vi "Host.vi"() -> ()   [LabVIEW 2018]
uses:
  <vilib>/userdefined/High Color/nirio_resource_hc.ctl
  <vilib>/vision/Image Controls.llb/IMAQ Image.ctl
  <instrlib>/niDCPower/nidcpower.llb/niDCPower Measurement Type.ctl
  <vilib>/FPGAPlugInAG/PXI-7953R/niLvFpga_Open_PXI-7953R.vi
  <vilib>/rvi/interface/common/dynamic/niFpgaDynamicAddResources.vi
  <vilib>/FPGAPlugInAG/Dynamic/niLvFpga_Reset_Dynamic.vi
  <vilib>/FPGAPlugInAG/Dynamic/niLvFpga_Run_Dynamic.vi
  <vilib>/Utility/error.llb/Error Cluster From Error Code.vi
  <vilib>/rvi/errors/niLvFpgaAdjustHostInterfaceError.vi
  <vilib>/FPGAPlugInAG/Dynamic/niLvFpga_Abort_Dynamic.vi
  <vilib>/rvi/interface/nirviOpenFPGA/nirviOpenFPGA.xnode
  FPGA Bitfiles/PelengCMV_FPGATarget_Target_uVRL8nzenuo.lvbitx
  <vilib>/rvi/interface/nirviMethod/nirviMethod.xnode
  <vilib>/rvi/interface/nirviReadWriteControl/nirviReadWriteControl.xnode
  NiFpgaLv.dll
  <vilib>/rvi/interface/Simulation/niFpgaSimulationCallBeginRW.vi
  <vilib>/FPGAPlugInAG/Dynamic/niLvFpga_ReadFifo_Dynamic.vi
  <vilib>/rvi/errors/niLvFpgaMergeErrorWithErrorCode.vi
panel:
  out "Waveform Chart 5":dbl(graph)=0.01180592873577935
  out "Waveform Chart 9":dbl(graph)=0.0007963780968987442
  out "Waveform Chart 7":dbl(graph)=0.08153866285805537
  out "Waveform Chart 6":dbl(graph)=-0.0005376097362887471
  out "Waveform Chart 4":dbl(graph)=0.015373157020534491
  out "Waveform Chart 3":dbl(graph)=-0.010436971741611662
  out "Waveform Chart 2":dbl(graph)=-0.0003554571679595278
  out "Тнак, мс":dbl
  in  "ПРОВЕРКА СБОЕВ?":bool=TRUE
  in  "ПРИМЕЧАНИЕ":string
  in  "Frames":path=path "C:/VPL/LabView_PRJ/ПЕЛЕНГ_CMV4000/FRAMES"
  in  "Светлый (T)\nТемный (F)":bool
  in  "SAVE":bool
  out "ПОСЛЕДНИЙ СБОЙ":string
  in  "МАСКИРУЕМ":i32[](array[numeric])=[0, 1, 2, 3, 4, 5, 6, 7, 8, 9, 10, 11, 12, 13, 14, 15, 16, 17, 18, 19, 20, 21, 22, 23, 24, 25, 26, 27, 28, 29, 30, 31, 32, 33, 34, 35, 36, 37, 38, 39, 40, 41, 42, 43, 44, 45, 46, 47, 48, 49, 50, 51, 52, 53, 54, 55, 56, 57, 58, 59, 60, 61, 62, 63, 64, 65, 66, 67, 68, 69, 70, 71, 72, 73, 74, 75, 76, 77, 78, 79, 80, 81, 82, 83, 84, 85, 86, 87, 88, 89, 90, 91, 92, 93, 94, 95, 96, 97, 98, 99, 100, 101, 102, 103, 104, 105, 106, 107, 108, 109, 110, 111, 112, 113, 114, 115, 116, 117, 118, 119, 120, 121, 122, 123, 124, 125, -1, -1, 0, 0, 0, 0, 0, 0, 0, 0, 0, 0, 0, 0, 0, 0, 0, 0, 0, 0, 0, 0, 0, 0, 0, 0, 0, 0, 0, 0, 0, 0, 0, 0, 0, 0, 0, 0, 0, 0, 0, 0, 0, 0, 0, 0, 0, 0, 0, 0, 0, 0, 0, 0, 0, 0, 0, 0, 0, 0, 0, 0, 0, 0, 0, 0, 0, 0, 0, 0, 0, 0, 0, 0, 0, 0, 0, 0, 0, 0, 0, 0, 0, 0, 0, 0, 0, 0, 0, 0, 0, 0, 0, 0, 0, 0, 0, 0, 0, 0, 0, 0, 0, 0, 0, 0, 0, 0, 0, 0, 0, 0, 0, 0, 0, 0, 0, 0, 0, 0, 0, 0, 0, 0, 0, 0, 0, 0, 0, 0]
  in  "НАДО":bool
  out "GC":u16
  in  "Непрерывно":bool
  out "Image":T1(plugin-control)
  in  "1":u8=1
  in  "2":u8=2
  in  "REQ_2":u8=7
  in  "REQ_1":u8=2
  in  "-1_прием":i8=-1
  out "Записали адресов":u32
  in  "9_прием":i8=9
  out "SPI_OUT":bool[](array[boolean])
  out "COUNT":u16
  out "D1":bool[](array[boolean])
  out "CONTROL":bool[](array[boolean])
  out "D9":bool[](array[boolean])
  out "T, C":dbl
  out "СБОЙ":string="ОК"
  in  "Запись всех регистров":u16[](array[numeric])=[0, 0, 8, 0, 0, 0, 0, 0, 0, 0, 0, 0, 0, 0, 0, 0, 0, 0, 0, 0, 0, 0, 0, 0, 0, 0, 0, 0, 0, 0, 0, 0, 0, 0, 0, 0, 0, 0, 0, 1, 0, 4, 0, 8, 0, 0, 0, 0, 1, 0, 0, 1, 0, 0, 1, 1, 0, 8, 0, 0, 0, 0, 1, 0, 0, 1, 0, 0, 1, 1, 1, 0, 3, 20, 8, 8, 8, 0, 85, 0, 255, 255, 3, 8, 4, 1, 14, 12, 64, 96, 96, 64, 96, 96, 101, 106, 96, 96, 96, 96, 0, 0, 3, 60, 8, 8, 8, 8, 0, 1, 0, 1, 0, 1, 3, 0, 9, 8, 1, 0, 0, 1, 0, 98, 0, 67]
  in  "SEU":path=path "C:/VPL/LabView_PRJ/ПЕЛЕНГ_CMV4000/LOGS/SEU"
  out "Сбои":i32
  in  "SEL_Time, мс":u32=100
  out "REG_WR":bool
  out "SEL":bool
  in  "For FIFO":i32=64
  in  "32768":u32=32768
  in  "Получить кадр":bool
  in  "VDD33_selcur":dbl=0.25 caption="current limit" format="%_6p"
  out "VDD33":i32
  out "VDD33":bool
  in  "SIM_SEL":bool
  in  "Облучаем?":bool
  in  "VDD20_selcur":dbl=0.2750000000000001 caption="current limit" format="%_6p"
  in  "VDDPIX_selcur":dbl=0.25000000000000006 caption="current limit" format="%_6p"
  in  "VRES_H_selcur":dbl=0.075 caption="current limit" format="%_6p"
  out "VDD20":i32
  out "VDD20":bool
  out "VDDPIX":i32=1
  out "VDDPIX":bool
  out "VRES_H":i32
  out "VRES_H":bool
  in  "REC(3,3V)":dbl=3.3 caption="voltage level" format="%_6p"
  in  "VDD20":dbl=5.0 caption="voltage level" format="%_6p"
  in  "VRES_H":dbl=5.0 caption="voltage level" format="%_6p"
  in  "REC_curlim":dbl=0.1 caption="current limit" format="%_6p"
  in  "FPGA+REP_curlim":dbl=0.5 caption="current limit" format="%_6p"
  in  "VDD20_curlim":dbl=0.30000000000000004 caption="current limit" format="%_6p"
  in  "VDD33_curlim":dbl=0.3 caption="current limit" format="%_6p"
  in  "VRES_H_curlim":dbl=0.1 caption="current limit" format="%_6p"
  out "REC_cur":dbl caption="measurement" format="%_6g"
  out "FPGA+REP_cur":dbl caption="measurement" format="%_6g"
  out "VDD20_cur":dbl caption="measurement" format="%_6g"
  out "VDD33_cur":dbl caption="measurement" format="%_6g"
  out "VRES_H_cur":dbl caption="measurement" format="%_6g"
  in  "FPGA+REP(6V)":dbl=5.0 caption="voltage level" format="%_6p"
  in  "VDD33":dbl=5.0 caption="voltage level" format="%_6p"
  in  "VDDPIX":dbl=5.0 caption="voltage level" format="%_6p"
  in  "VDDPIX_curlim":dbl=0.30000000000000004 caption="current limit" format="%_6p"
  out "VDDPIX_cur":dbl caption="measurement" format="%_6g"
  in  "TH_RES_curlim":dbl=0.2 caption="current limit" format="%_6p"
  out "TH_RES_cur":dbl caption="measurement" format="%_6g"
  in  "TH_RES":dbl=-20.0 caption="voltage level" format="%_6p"
  in  "Грелка":bool
  in  "Питание":bool
  in  "Стоп":bool
  in  "REC_FPGA_TH":refnum<k15>="PXI1Slot4" caption="instrument handle"
  in  "PIX_20":refnum<k15>="PXI1Slot2" caption="instrument handle"
  in  "33_RES":refnum<k15>="PXI1Slot3" caption="instrument handle"
  in  "resource name":T2="RIO0"
  in  "SEL":path=path "C:/VPL/LabView_PRJ/ПЕЛЕНГ_CMV4000/LOGS/SEL"
  out "Номер образца":string="1"
  out "Температура":string="25"
  out "Data":u32[][](array[numeric])
  out "Image Out":T1
  out "СБОЙ!":bool
  # "ЧТОБЫ ЗАМАСКИРОВАТЬ, ПОМЕНЯЙ НОМЕР РЕГИСТРА НА -1"
  # "КАЖДОЕ ВЫКЛЮЧЕНИЕ СОПРОВОЖДАЕТСЯ 300МС ЗАДЕРЖКОЙ"
  # "43 регистр\n8 = 53мс\n15 = 100мс\n30 = 200мс\n76 = 500мс\n152 = 1000мс\n227 = 1500мс"
  # "ЕСЛИ ХОЧЕШЬ СНЯТЬ ПРИ РАЗНЫХ ВРЕМЕНАХ НАКОПЛЕНИЯ, ТО ОТКЛЮЧИ ПРОВЕРКУ РЕГИСТРОВ И МЕНЯЙ ЗНАЧЕНИЕ В РЕГСИРЕ 43!"
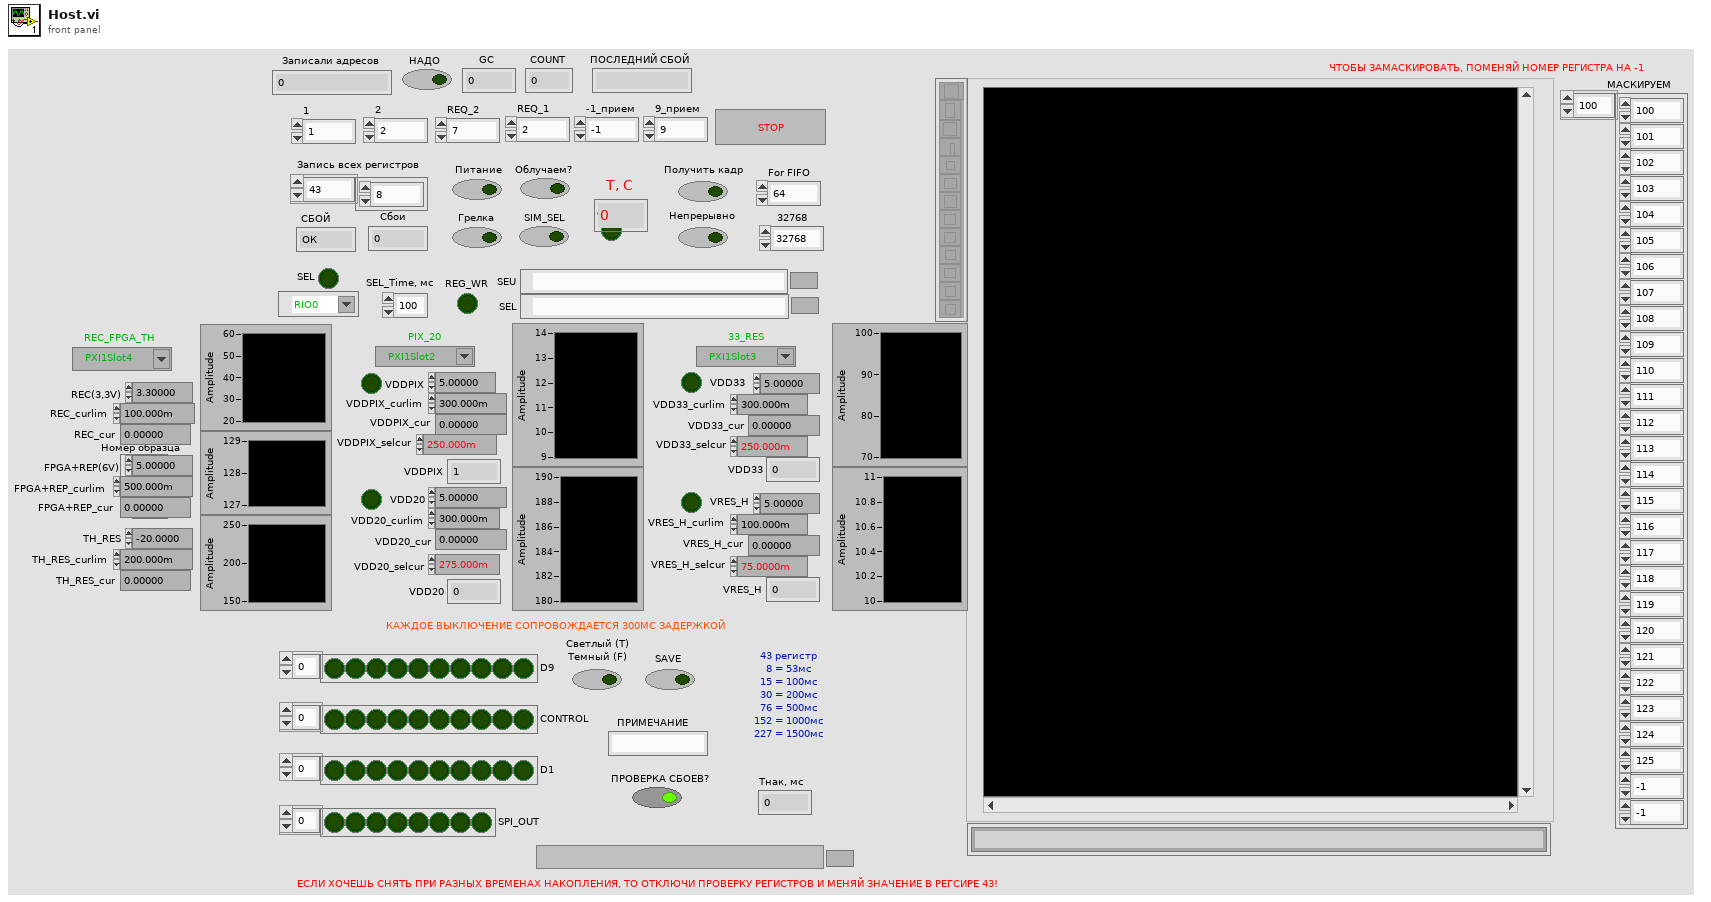
[diagram p1: front panel]
types:
  T1 = typedef "IMAQ Image.ctl" = refnum<image>
  T2 = typedef "nirio_resource_hc.ctl" = tag
  T3 = typedef "Image Type" = u32
  T4 = enum16{"open", "replace", "create", "open or create", "replace or create", "replace or create with confirmation"}
  T5 = typedef "niDCPower Measurement Type.ctl" = i32
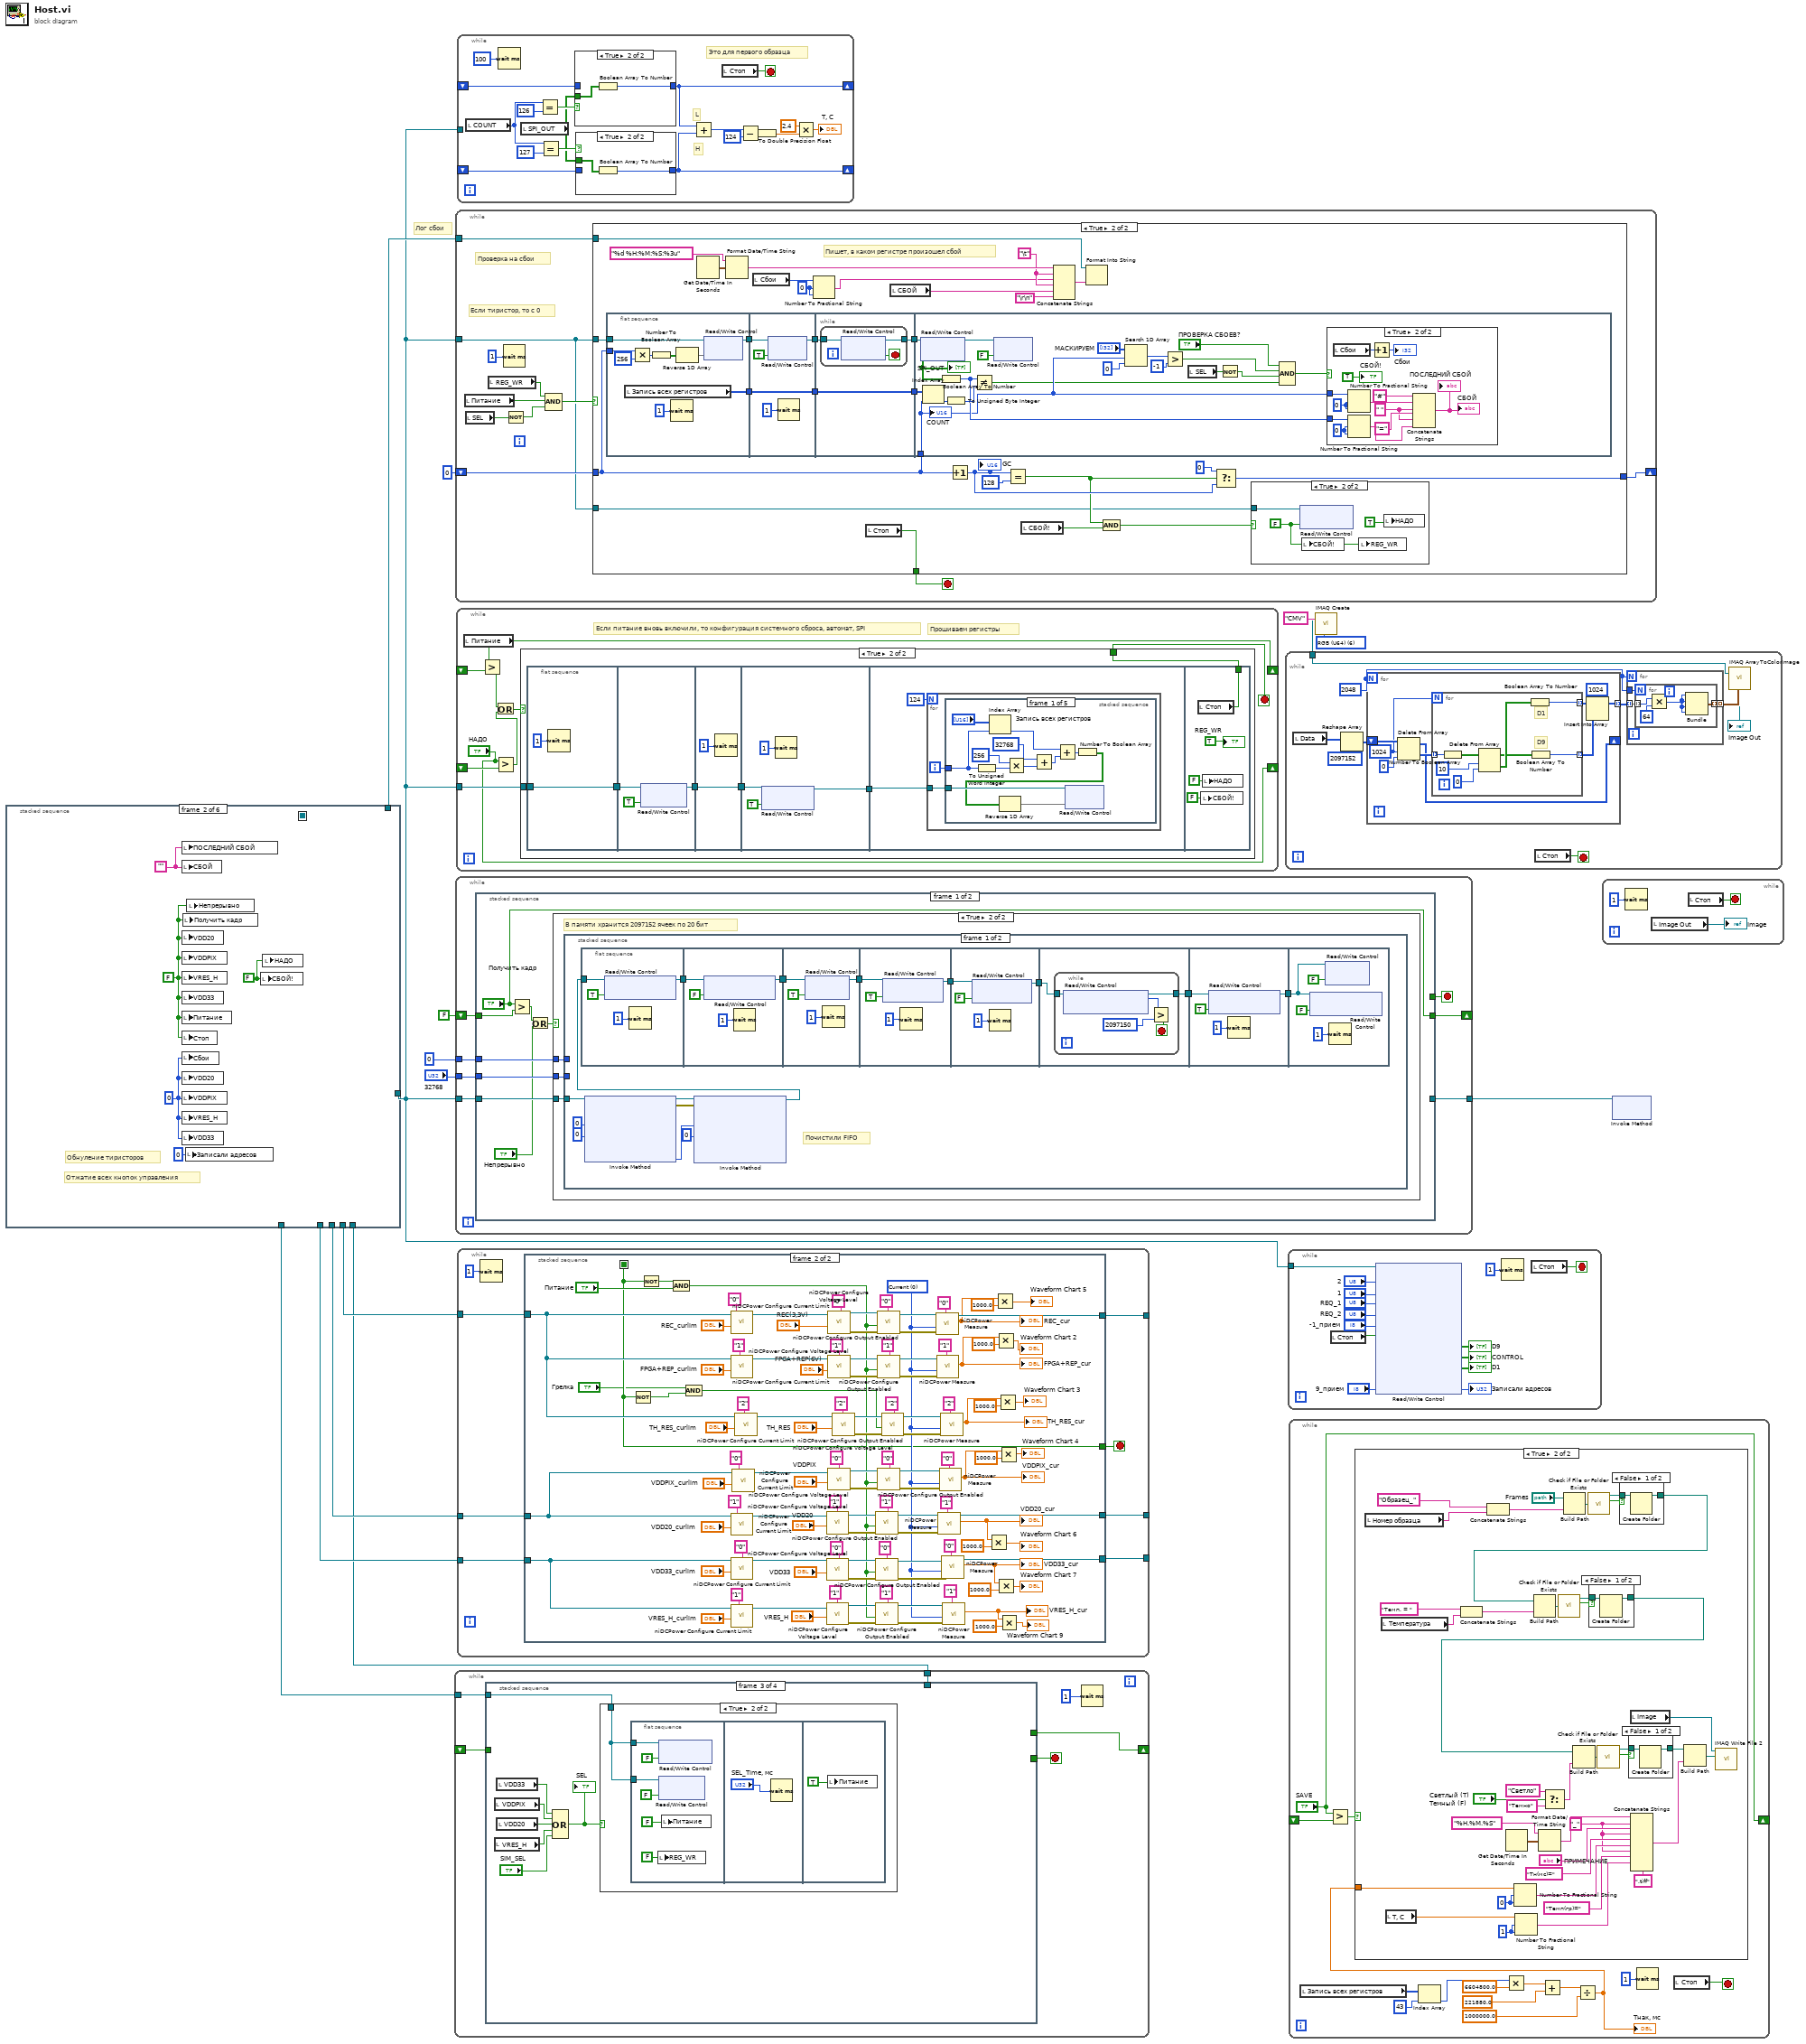
[diagram p0: block diagram]
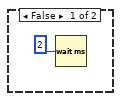
[diagram p8: hidden frame]
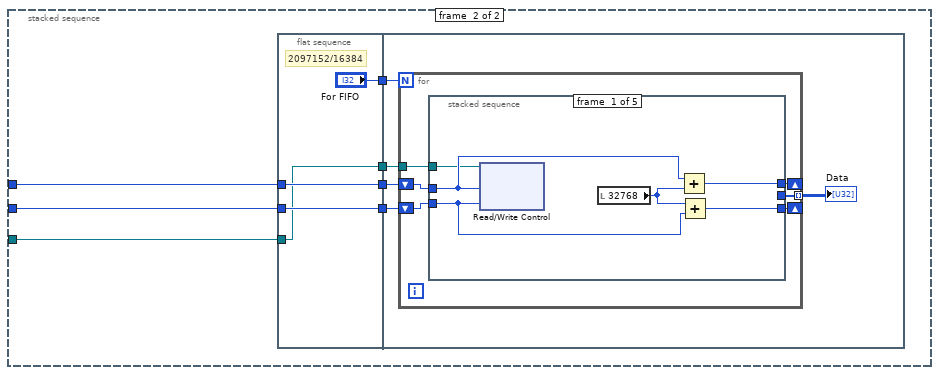
[diagram p9: hidden frame]
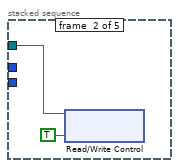
[diagram p10: hidden frame]
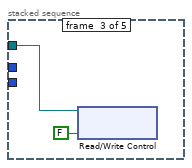
[diagram p11: hidden frame]
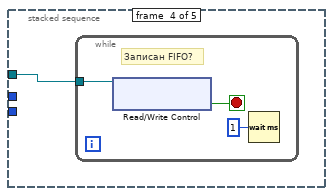
[diagram p12: hidden frame]
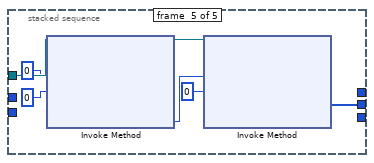
[diagram p13: hidden frame]
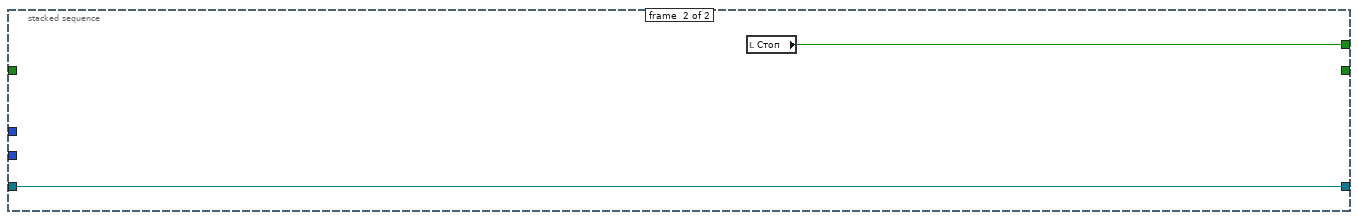
[diagram p14: hidden frame]
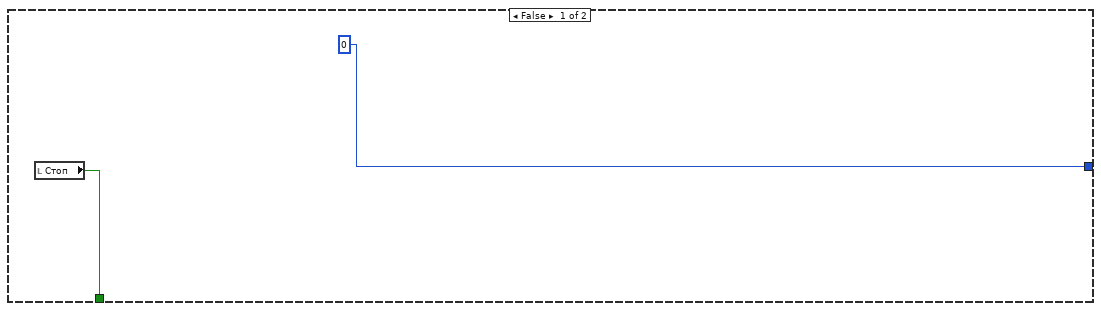
[diagram p15: hidden frame]
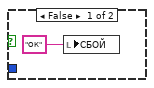
[diagram p17: hidden frame]
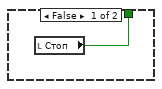
[diagram p18: hidden frame]
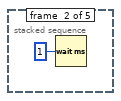
[diagram p19: hidden frame]
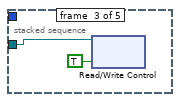
[diagram p20: hidden frame]
diagram:
  w3 = T3 6 items=["Grayscale (U8)", "Grayscale (I16)", "Grayscale (SGL)", "Complex (CSG)", "RGB (U32)", "HSL (U32)", "RGB (U64)"] ("Image Type")
  # "Лог сбои"
  n1 = stacked-sequence {
    seq-local: [_ _ _ _ w106 _] -> [_ _ _ _ _ w114]
    tunnel: [_ _ _ _ w106 _] -> w5
    tunnel: [_ _ _ _ _ w117] -> w13
    tunnel: [_ _ _ _ _ w116] -> w14
    tunnel: [_ _ _ _ _ w115] -> w15
    tunnel: [_ _ w29 _ _ _] -> w12
    tunnel: [_ _ _ _ w106 _] -> w10
    tunnel: [_ _ _ w68 _ _] -> w9
    frame #0 {
      n2 = call "Begin.vi"() -> ("Температура 2"=→"Температура":string, "Номер образца 2"=→"Номер образца":string)  [unwired: 10 in]
    }
    frame #1 {
      w22 = FALSE ("СБОЙ!")
      w19 = 0
      w20 = ""
      w21 = FALSE
      # "Обнуление тиристоров"
      # "Отжатие всех кнопок управления"
      n3 = local write "ПОСЛЕДНИЙ СБОЙ"(w20) -> ()
      n4 = local write "СБОЙ"(w20) -> ()
      n5 = local write "VDD20"(w21) -> ()
      n6 = local write "VDDPIX"(w21) -> ()
      n7 = local write "VRES_H"(w21) -> ()
      n8 = local write "VDD33"(w21) -> ()
      n9 = local write "Питание"(w21) -> ()
      n10 = local write "Стоп"(w21) -> ()
      n11 = local write "Сбои"(w19) -> ()
      n12 = local write "VDD20"(w19) -> ()
      n13 = local write "VDDPIX"(w19) -> ()
      n14 = local write "VRES_H"(w19) -> ()
      n15 = local write "VDD33"(w19) -> ()
      n16 = local write "Получить кадр"(w21) -> ()
      n17 = local write "Записали адресов"(u32 0 ("Записали адресов")) -> ()
      n18 = local write "Непрерывно"(w21) -> ()
      n19 = local write "СБОЙ!"(w22) -> ()
      n20 = local write "НАДО"(w22) -> ()
    }
    frame #2 {
      w32 = "\t"
      # "Инициализаци первой строки лога по токам"
      n21 = local read "Номер образца"() -> (w53:string)
      n22 = Build Path(base path="SEL", name or relative path=w53) -> (appended path=w55:path)
      n23 = Get Date/Time In Seconds() -> (seconds since 1Jan1904=w45:timestamp)
      n24 = call <vilib>:"Check if File or Folder Exists.vi"("path"=w55) -> ("file or folder exists?"=w56:bool, "dup path"=w57:path)  [unwired: 8 in, 1 out]
      n25 = Format Date/Time String(time format string (%c)="%d %H.%M.%S", seconds (now)=w45) -> (date/time string=w42:string)  [unwired: 1 in]
      n26 = case shown="False" w56 {
        tunnel: w57 -> [w66 w67]
        tunnel: [w65 w67] -> w51
        frame False {
          n27 = Create Folder(path (use dialog)=w66) -> (created path=w65:path)  [unwired: 2 in, 2 out]
        }
        frame True {
        }
      }
      n28 = local read "Температура"() -> (w50:string)
      n29 = Concatenate Strings(w42, ".xls" ("string")) -> (w40:string)
      n30 = Build Path(base path=w51, name or relative path=w50) -> (appended path=w31:path)
      n31 = call <vilib>:"Check if File or Folder Exists.vi"("path"=w31) -> ("file or folder exists?"=w30:bool, "dup path"=w52:path)  [unwired: 8 in, 1 out]
      n32 = case shown="False" w30 {
        tunnel: w52 -> [w63 w64]
        tunnel: [w62 w64] -> w39
        frame False {
          n33 = Create Folder(path (use dialog)=w63) -> (created path=w62:path)  [unwired: 2 in, 2 out]
        }
        frame True {
        }
      }
      n34 = Build Path(base path=w39, name or relative path=w40) -> (appended path=w43:path)
      n35 = Open/Create/Replace File(file path (use dialog)=w43, operation (0:open)=T4."open or create", access (0:read/write)=enum16{"read/write", "read-only", "write-only"}."read/write") -> (refnum out=w46:refnum<file>)  [unwired: 3 in, 2 out]
      n36 = case shown="True" TRUE {
        tunnel: w46 -> [w58 w61]
        tunnel: [w58 w59] -> w38
        frame False {
        }
        frame True {
          n37 = Set File Position(refnum=w61, from (0:start)=enum16{"start", "end", "current"}."end") -> (refnum out=w59:refnum<file>)  [unwired: 2 in, 1 out]
        }
      }
      n38 = Format Into String(initial string=w38, "Time" ("input 1"), w32, "VDD20_cur" ("input 1"), w32, "VDDPIX_cur" ("input 1"), w32, "VRES_H_cur" ("input 1"), w32, "VDD33_cur" ("input 1"), w32, "VDD20_sel" ("input 1"), w32, "VDDPIX_sel" ("input 1"), w32, "VRES_H_sel" ("input 1"), w32, "VDD33_sel" ("input 1"), w32, "Облучение" ("input 1"), "\r\n") -> (resulting string=w29:refnum<file>)  [unwired: 2 in, 1 out]
    }
    frame #3 {
      w77 = "\t"
      n39 = local read "Номер образца"() -> (w91:string)
      n40 = Build Path(base path="SEU", name or relative path=w91) -> (appended path=w93:path)
      n41 = Get Date/Time In Seconds() -> (seconds since 1Jan1904=w86:timestamp)
      n42 = call <vilib>:"Check if File or Folder Exists.vi"("path"=w93) -> ("file or folder exists?"=w94:bool, "dup path"=w95:path)  [unwired: 8 in, 1 out]
      n43 = Format Date/Time String(time format string (%c)="%d %H.%M.%S", seconds (now)=w86) -> (date/time string=w84:string)  [unwired: 1 in]
      n44 = case shown="False" w94 {
        tunnel: w95 -> [w104 w105]
        tunnel: [w103 w105] -> w89
        frame False {
          n45 = Create Folder(path (use dialog)=w104) -> (created path=w103:path)  [unwired: 2 in, 2 out]
        }
        frame True {
        }
      }
      n46 = local read "Температура"() -> (w88:string)
      n47 = Concatenate Strings(w84, ".xls" ("string")) -> (w83:string)
      n48 = Build Path(base path=w89, name or relative path=w88) -> (appended path=w80:path)
      n49 = call <vilib>:"Check if File or Folder Exists.vi"("path"=w80) -> ("file or folder exists?"=w79:bool, "dup path"=w90:path)  [unwired: 8 in, 1 out]
      n50 = case shown="False" w79 {
        tunnel: w90 -> [w101 w102]
        tunnel: [w100 w102] -> w82
        frame False {
          n51 = Create Folder(path (use dialog)=w101) -> (created path=w100:path)  [unwired: 2 in, 2 out]
        }
        frame True {
        }
      }
      n52 = Build Path(base path=w82, name or relative path=w83) -> (appended path=w85:path)
      n53 = Open/Create/Replace File(file path (use dialog)=w85, operation (0:open)=T4."open or create", access (0:read/write)=enum16{"read/write", "read-only", "write-only"}."read/write") -> (refnum out=w87:refnum<file>)  [unwired: 3 in, 2 out]
      n54 = case shown="True" TRUE {
        tunnel: w87 -> [w96 w99]
        tunnel: [w96 w97] -> w81
        frame False {
        }
        frame True {
          n55 = Set File Position(refnum=w99, from (0:start)=enum16{"start", "end", "current"}."end") -> (refnum out=w97:refnum<file>)  [unwired: 2 in, 1 out]
        }
      }
      n56 = Format Into String(initial string=w81, "Time" ("input 1"), w77, "Count" ("input 3"), w77, "#reg" ("input 5"), "\r\n") -> (resulting string=w68:refnum<file>)  [unwired: 2 in, 1 out]
    }
    frame #4 {
      n57 = xnode "Open FPGA VI Reference"("resource name"="resource name") -> ("FPGA VI Reference Out"=w111:refnum<k20>, "error out"=w109:errorcluster)  [unwired: 1 in]
      n58 = xnode "Invoke Method"("FPGA VI Reference In"=w111, "error in"=w109) -> ("FPGA VI Reference Out"=w108:refnum<k20>, "error out"=w110:errorcluster)
      n59 = xnode "Invoke Method"("FPGA VI Reference In"=w108, "error in"=w110) -> ("FPGA VI Reference Out"=w106:refnum<k20>)  [unwired: 1 in, 1 out]
    }
    frame #5 {
      w112 = FALSE ("SYS_RESET")
      n60 = xnode "Read/Write Control"("FPGA VI Reference In"=w114, "SYS_RESET"=w112, "Стоп"=w112, "Данные"=w112, "FRAME_REQ"=w112, "Конец анализа"=w112) -> ()  [unwired: 1 in, 2 out]
      n61 = local write "REG_WR"(FALSE ("Прошили регистры")) -> ()
      n62 = call <instrlib>:"niDCPower Initialize.vi"("resource name"="REC_FPGA_TH") -> ("error out"=w127:errorcluster, "instrument handle out"=w130:refnum<k15>)  [unwired: 3 in, 6 out]
      n63 = call <instrlib>:"niDCPower Initialize.vi"("resource name"="PIX_20") -> ("error out"=w128:errorcluster, "instrument handle out"=w131:refnum<k15>)  [unwired: 3 in, 6 out]
      n64 = call <instrlib>:"niDCPower Initialize.vi"("resource name"="33_RES") -> ("error out"=w129:errorcluster, "instrument handle out"=w132:refnum<k15>)  [unwired: 3 in, 6 out]
      n65 = call <instrlib>:"niDCPower Configure Voltage Level.vi"("error in (no error)"=w127, "voltage level"=0.0, "channel name"="0,1,2", "instrument handle"=w130) -> ("instrument handle out"=w115:refnum<k15>)  [unwired: 6 in, 1 out]
      n66 = call <instrlib>:"niDCPower Configure Voltage Level.vi"("error in (no error)"=w128, "voltage level"=0.0, "channel name"="0,1", "instrument handle"=w131) -> ("instrument handle out"=w116:refnum<k15>)  [unwired: 6 in, 1 out]
      n67 = call <instrlib>:"niDCPower Configure Voltage Level.vi"("error in (no error)"=w129, "voltage level"=0.0, "channel name"="0,1", "instrument handle"=w132) -> ("instrument handle out"=w117:refnum<k15>)  [unwired: 6 in, 1 out]
    }
  }
  n68 = while {
    tunnel: w12 -> [w137]
    shift-right: [w136] -> _
    shift-left: _ -> [w135]
    tunnel: w10 -> [w133]
    stop <- w134 stop-if-true
    n69 = stacked-sequence {
      tunnel: w137 -> [_ w200 _ _]
      tunnel: [w141 _ _ _] -> w136
      tunnel: w135 -> [w139 _ _ _]
      tunnel: [_ _ _ w224] -> w134
      tunnel: w133 -> [_ _ w207 w222]
      frame #0 {
        # "Проверка токов на тиристоры"
        n70 = local read "Питание"() -> (w141:bool)
        n71 = flat-sequence {
          tunnel: w140 -> [w142]
          frame #0 {
            n72 = case shown="True" w142 {
              frame False {
              }
              frame True {
                n73 = Wait (ms)(milliseconds to wait=u32 300) -> ()  [unwired: 1 out]
              }
            }
          }
          frame #1 {
            n74 = local read "VDD33_cur"() -> (w144:dbl)
            n75 = local read "VRES_H_cur"() -> (w149:dbl)
            n76 = local read "VDDPIX_cur"() -> (w152:dbl)
            n77 = local read "VDD20_cur"() -> (w155:dbl)
            n78 = Greater?(x=w144, y="VDD33_selcur") -> (0:w146:bool)
            "VDD33" <- w146
            n79 = Greater?(x=w149, y="VRES_H_selcur") -> (0:w147:bool)
            "VRES_H" <- w147
            n80 = Greater?(x=w155, y="VDD20_selcur") -> (0:w153:bool)
            "VDD20" <- w153
            n81 = Greater?(x=w152, y="VDDPIX_selcur") -> (0:w150:bool)
            "VDDPIX" <- w150
            n82 = case shown="True" w146 {
              frame False {
              }
              frame True {
                n83 = local read "VDD33"() -> (w157:i32)
                n84 = Increment(x=w157) -> (x+1=→"VDD33":i32)
              }
            }
            n85 = case shown="True" w153 {
              frame False {
              }
              frame True {
                n86 = local read "VDD20"() -> (w163:i32)
                n87 = Increment(x=w163) -> (x+1=→"VDD20":i32)
              }
            }
            n88 = case shown="True" w150 {
              frame False {
              }
              frame True {
                n89 = local read "VDDPIX"() -> (w160:i32)
                n90 = Increment(x=w160) -> (x+1=→"VDDPIX":i32)
              }
            }
            n91 = case shown="True" w147 {
              frame False {
              }
              frame True {
                n92 = local read "VRES_H"() -> (w159:i32)
                n93 = Increment(x=w159) -> (x+1=→"VRES_H":i32)
              }
            }
          }
        }
        n94 = Greater?(x=w141, y=w139) -> (0:w140:bool)
      }
      frame #1 {
        w166 = i16 2 ("precision (6)")
        w185 = i16 0 ("width (-)")
        w190 = i16 3 ("width (-)")
        w169 = "\t"
        n95 = local read "VDDPIX_cur"() -> (w188:dbl)
        n96 = local read "VRES_H_cur"() -> (w187:dbl)
        n97 = local read "VDD20_cur"() -> (w189:dbl)
        n98 = local read "VDD33_cur"() -> (w186:dbl)
        n99 = local read "VDDPIX"() -> (w183:i32)
        n100 = local read "VRES_H"() -> (w182:i32)
        n101 = local read "VDD20"() -> (w184:i32)
        n102 = local read "VDD33"() -> (w181:i32)
        n103 = Number To Fractional String(number=w189, width (-)=w190, precision (6)=w190) -> (F-format string=w180:string)  [unwired: 1 in]
        n104 = Number To Fractional String(number=w188, width (-)=w190, precision (6)=w190) -> (F-format string=w179:string)  [unwired: 1 in]
        n105 = Number To Fractional String(number=w187, width (-)=w190, precision (6)=w190) -> (F-format string=w178:string)  [unwired: 1 in]
        n106 = Number To Fractional String(number=w186, width (-)=w190, precision (6)=w190) -> (F-format string=w177:string)  [unwired: 1 in]
        n107 = Number To Fractional String(number=w184, width (-)=w185, precision (6)=w185) -> (F-format string=w176:string)  [unwired: 1 in]
        n108 = Number To Fractional String(number=w183, width (-)=w185, precision (6)=w185) -> (F-format string=w175:string)  [unwired: 1 in]
        n109 = Number To Fractional String(number=w182, width (-)=w185, precision (6)=w185) -> (F-format string=w174:string)  [unwired: 1 in]
        n110 = Number To Fractional String(number=w181, width (-)=w185, precision (6)=w185) -> (F-format string=w173:string)  [unwired: 1 in]
        n111 = Get Date/Time In Seconds() -> (seconds since 1Jan1904=w205:timestamp)
        n112 = Format Date/Time String(time format string (%c)="%d %H:%M:%S:%3u", seconds (now)=w205) -> (date/time string=w191:string)  [unwired: 1 in]
        n113 = local read "VDD33"() -> (w196:bool)
        n114 = local read "VDDPIX"() -> (w195:bool)
        n115 = local read "VDD20"() -> (w194:bool)
        n116 = local read "VRES_H"() -> (w193:bool)
        n117 = local read "SIM_SEL"() -> (w192:bool)
        n118 = Compound Arithmetic op=OR(w196, w195, w194, w193, w192) -> (w172:bool)
        n119 = Select(t="О", s="Облучаем?", f="") -> (s? t:f=w171:string)
        n120 = Select(t="!!!", s=w172, f="") -> (s? t:f=w170:string)
        n121 = local read "T, C"() -> (w167:dbl)
        n122 = Number To Fractional String(number=w167, width (-)=w166, precision (6)=w166) -> (F-format string=w165:string)  [unwired: 1 in]
        n123 = Concatenate Strings(w191, w169, w180, w169, w179, w169, w178, w169, w177, w169, w176, w169, w175, w169, w174, w169, w173, w169, w171, w169, w170, w169, "Т = ", w165, "\r\n") -> (w204:string)
        n124 = Format Into String(initial string=w200, w204) -> ()  [unwired: 2 in, 2 out]
      }
      frame #2 {
        n125 = local read "VDDPIX"() -> (w211:bool)
        n126 = local read "VRES_H"() -> (w209:bool)
        n127 = local read "VDD33"() -> (w212:bool)
        n128 = local read "VDD20"() -> (w210:bool)
        n129 = Compound Arithmetic op=OR(w212, w211, w210, w209, "SIM_SEL") -> (w206:bool)
        "SEL" <- w206
        n130 = case shown="True" w206 {
          tunnel: w207 -> [_ w213]
          frame False {
          }
          frame True {
            n131 = flat-sequence {
              tunnel: w213 -> [w218]
              tunnel: w213 -> [w217]
              frame #0 {
                n132 = local write "REG_WR"(FALSE ("SYS_RESET")) -> ()
                n133 = xnode "Read/Write Control"("FPGA VI Reference In"=w217, "Автомат"=FALSE ("SYS_RESET")) -> ()  [unwired: 1 in, 2 out]
                n134 = xnode "Read/Write Control"("FPGA VI Reference In"=w218, "SYS_RESET"=FALSE) -> ()  [unwired: 1 in, 2 out]
                n135 = local write "Питание"(FALSE ("SYS_RESET")) -> ()
              }
              frame #1 {
                n136 = Wait (ms)(milliseconds to wait="SEL_Time, мс") -> ()  [unwired: 1 out]
              }
              frame #2 {
                n137 = local write "Питание"(TRUE ("SYS_RESET")) -> ()
              }
            }
          }
        }
      }
      frame #3 {
        n138 = local read "Питание"() -> (w223:bool)
        n139 = case shown="False" w223 {
          tunnel: w222 -> [w226 _]
          frame False {
            w225 = FALSE
            n140 = xnode "Read/Write Control"("FPGA VI Reference In"=w226, "SYS_RESET"=w225) -> ()  [unwired: 1 in, 2 out]
            n141 = xnode "Read/Write Control"("FPGA VI Reference In"=w226, "Автомат"=w225) -> ()  [unwired: 1 in, 2 out]
            n142 = local write "REG_WR"(w225) -> ()
          }
          frame True {
          }
        }
        n143 = local read "Стоп"() -> (w224:bool)
      }
    }
    n144 = Wait (ms)(milliseconds to wait=u32 1) -> ()  [unwired: 1 out]
  }
  n145 = while {
    tunnel: w5 -> [w227]
    tunnel: w9 -> [w229]
    shift-right: [w230] -> _
    shift-left: u16 0 -> [w231]
    stop <- w228 stop-if-true
    # "Проверка на сбои"
    # "Если тиристор, то с 0"
    n146 = local read "Питание"() -> (w236:bool)
    n147 = local read "SEL"() -> (w234:bool)
    n148 = local read "REG_WR"() -> (w237:bool)
    n149 = Wait (ms)(milliseconds to wait=u32 1) -> ()  [unwired: 1 out]
    n150 = Not(x=w234) -> (.not. x?=w233:bool)
    n151 = Compound Arithmetic op=AND(w237, w236, w233) -> (w235:bool)
    n152 = case shown="True" w235 {
      tunnel: w231 -> [_ w261]
      tunnel: [u8 0 w266] -> w230
      tunnel: w227 -> [_ w265]
      tunnel: w229 -> [_ w254]
      tunnel: [w238 w245] -> w228
      tunnel: w227 -> [_ w240]
      frame False {
        n153 = local read "Стоп"() -> (w238:bool)
      }
      frame True {
        w250 = i16 0 ("width (-)")
        w252 = "\t"
        # "Пишет, в каком регистре произошел сбой"
        n154 = flat-sequence {
          tunnel: w261 -> [w279]
          tunnel: w265 -> [w274]
          tunnel: [w273] -> w264
          tunnel: [w272] -> w258
          tunnel: w264 -> [w284]
          tunnel: [w281] -> w263
          tunnel: [w280] -> w259
          tunnel: w258 -> [w280]
          tunnel: w263 -> [w287]
          tunnel: [w286] -> w262
          tunnel: [w285] -> w260
          tunnel: w259 -> [w285]
          tunnel: w262 -> [w309]
          tunnel: w261 -> [w297]
          tunnel: w260 -> [w308]
          frame #0 {
            n155 = local read "Запись всех регистров"() -> (w272:u16[])
            n156 = Multiply(x=w279, y=u16 256) -> (x*y=w276:u16)
            n157 = Number To Boolean Array(number=w276) -> (Boolean array=w277:bool[])
            n158 = Wait (ms)(milliseconds to wait=u32 1) -> ()  [unwired: 1 out]
            n159 = Reverse 1D Array(array=w277) -> (reversed array=w275:bool[])
            n160 = xnode "Read/Write Control"("FPGA VI Reference In"=w274, "SPI_IN"=w275) -> ("FPGA VI Reference Out"=w273:refnum<k20>)  [unwired: 1 in, 1 out]
          }
          frame #1 {
            n161 = xnode "Read/Write Control"("FPGA VI Reference In"=w284, "SPI"=TRUE) -> ("FPGA VI Reference Out"=w281:refnum<k20>)  [unwired: 1 in, 1 out]
            n162 = Wait (ms)(milliseconds to wait=u32 1) -> ()  [unwired: 1 out]
          }
          frame #2 {
            n163 = while {
              tunnel: w287 -> [w290]
              tunnel: [w288] -> w286
              stop <- w289 stop-if-true
              n164 = xnode "Read/Write Control"("FPGA VI Reference In"=w290) -> ("FPGA VI Reference Out"=w288:refnum<k20>, "SPI_OFF"=w289:bool)  [unwired: 1 in, 1 out]
            }
          }
          frame #3 {
            n165 = xnode "Read/Write Control"("FPGA VI Reference In"=w309) -> ("FPGA VI Reference Out"=w304:refnum<k20>, "SPI_OUT"=w307:bool[])  [unwired: 1 in, 1 out]
            "SPI_OUT" <- w307
            n166 = Index Array(array=w308, index=w297) -> (element=w306:u16)
            n167 = Boolean Array To Number(Boolean array=w307) -> (number=w302:u8)
            n168 = To Unsigned Byte Integer(number=w306) -> (unsigned 8bit integer=w305:u8)
            n169 = Not Equal?(x=w302, y=w305) -> (x != y?=w292:bool)
            n170 = xnode "Read/Write Control"("FPGA VI Reference In"=w304, "SPI"=FALSE) -> ()  [unwired: 1 in, 2 out]
            n171 = Search 1D Array(1D array="МАСКИРУЕМ", element=w297, start index (0)=0) -> (index of element=w298:i32)
            n172 = Greater?(x=w298, y=-1) -> (0:w294:bool)
            n173 = local read "SEL"() -> (w296:bool)
            n174 = Not(x=w296) -> (.not. x?=w293:bool)
            n175 = Compound Arithmetic op=AND("ПРОВЕРКА СБОЕВ?", w294, w293, w292) -> (w291:bool)
            n176 = case shown="True" w291 {
              tunnel: w297 -> [_ w315]
              tunnel: w302 -> [_ w314]
              frame False {
                n177 = local write "СБОЙ"("ОК" ("Где сбой")) -> ()
              }
              frame True {
                w311 = " " ("string")
                w320 = i16 0 ("width (-)")
                w321 = i16 0 ("width (-)")
                n178 = local read "Сбои"() -> (w323:i32)
                n179 = Number To Fractional String(number=w315, width (-)=w321, precision (6)=w321) -> (F-format string=w318:string)  [unwired: 1 in]
                n180 = Number To Fractional String(number=w314, width (-)=w320, precision (6)=w320) -> (F-format string=w312:string)  [unwired: 1 in]
                n181 = Increment(x=w323) -> (x+1=→"Сбои":i32)
                n182 = Concatenate Strings("#" ("string"), w318, w311, "=" ("string"), w311, w312) -> (→"СБОЙ" →"ПОСЛЕДНИЙ СБОЙ":string)
                "СБОЙ!" <- TRUE ("СБОЙ!")
              }
            }
            "COUNT" <- w297
          }
        }
        n183 = Get Date/Time In Seconds() -> (seconds since 1Jan1904=w257:timestamp)
        n184 = Format Date/Time String(time format string (%c)="%d %H:%M:%S:%3u", seconds (now)=w257) -> (date/time string=w255:string)  [unwired: 1 in]
        n185 = local read "Сбои"() -> (w249:i32)
        n186 = Number To Fractional String(number=w249, width (-)=w250, precision (6)=w250) -> (F-format string=w248:string)  [unwired: 1 in]
        n187 = local read "Стоп"() -> (w245:bool)
        n188 = local read "СБОЙ"() -> (w247:string)
        n189 = Increment(x=w261) -> (x+1=w246:u16)
        "GC" <- w246
        n190 = Equal?(x=w246, y=u16 128) -> (x = y?=w243:bool)
        n191 = local read "СБОЙ!"() -> (w242:bool)
        n192 = Concatenate Strings(w255, w252, w248, w252, w247, "\r\n") -> (w253:string)
        n193 = Format Into String(initial string=w254, w253) -> ()  [unwired: 2 in, 2 out]
        n194 = And(x=w243, y=w242) -> (x .and. y?=w241:bool)
        n195 = Select(t=u16 0, s=w243, f=w246) -> (s? t:f=w266:u16)
        n196 = case shown="True" w241 {
          tunnel: w240 -> [_ w270]
          frame False {
          }
          frame True {
            w269 = FALSE ("SYS_RESET")
            n197 = xnode "Read/Write Control"("FPGA VI Reference In"=w270, "SYS_RESET"=w269) -> ()  [unwired: 1 in, 2 out]
            n198 = local write "СБОЙ!"(w269) -> ()
            n199 = local write "REG_WR"(w269) -> ()
            n200 = local write "НАДО"(TRUE ("НАДО")) -> ()
          }
        }
      }
    }
  }
  n201 = while {
    tunnel: w5 -> [w330]
    tunnel: [w329] -> w11
    tunnel: "32768" -> [w328]
    tunnel: u32 0 -> [w326]
    shift-right: [w324] -> _
    shift-left: FALSE ("Получить кадр") -> [w325]
    stop <- w327 stop-if-true
    n202 = stacked-sequence {
      tunnel: w330 -> [w337 w437]
      tunnel: [_ w437] -> w329
      tunnel: w328 -> [w338 _]
      tunnel: [_ w436] -> w327
      tunnel: w326 -> [w336 _]
      tunnel: w325 -> [w335 _]
      tunnel: ["Получить кадр" _] -> w324
      frame #0 {
        n203 = Greater?(x="Получить кадр", y=w335) -> (0:w334:bool)
        n204 = Or(x=w334, y="Непрерывно") -> (x .or. y?=w332:bool)
        n205 = case shown="True" w332 {
          tunnel: w337 -> [_ w342]
          tunnel: w338 -> [_ w341]
          tunnel: w336 -> [_ w340]
          frame False {
            n206 = Wait (ms)(milliseconds to wait=u32 2) -> ()  [unwired: 1 out]
          }
          frame True {
            # "В памяти хранится 2097152 ячеек по 20 бит"
            n207 = stacked-sequence {
              tunnel: w342 -> [w346 w399]
              tunnel: w341 -> [_ w395]
              tunnel: w340 -> [_ w397]
              frame #0 {
                # "Почистили FIFO"
                n208 = flat-sequence {
                  tunnel: w345 -> [w361]
                  tunnel: [w360] -> w349
                  tunnel: [w365] -> w350
                  tunnel: w349 -> [w364]
                  tunnel: w350 -> [w367]
                  tunnel: [w366] -> w348
                  tunnel: [w371] -> w351
                  tunnel: w348 -> [w370]
                  tunnel: w351 -> [w375]
                  tunnel: [w374] -> w347
                  tunnel: w347 -> [w379]
                  tunnel: [w378] -> w344
                  tunnel: w344 -> [w386]
                  tunnel: [w385] -> w343
                  tunnel: w343 -> [w389]
                  frame #0 {
                    n209 = xnode "Read/Write Control"("FPGA VI Reference In"=w361, "Конец анализа"=TRUE) -> ("FPGA VI Reference Out"=w360:refnum<k20>)  [unwired: 1 in, 1 out]
                    n210 = Wait (ms)(milliseconds to wait=u32 1) -> ()  [unwired: 1 out]
                  }
                  frame #1 {
                    n211 = xnode "Read/Write Control"("FPGA VI Reference In"=w364, "Конец анализа"=FALSE) -> ("FPGA VI Reference Out"=w365:refnum<k20>)  [unwired: 1 in, 1 out]
                    n212 = Wait (ms)(milliseconds to wait=u32 1) -> ()  [unwired: 1 out]
                  }
                  frame #2 {
                    n213 = xnode "Read/Write Control"("FPGA VI Reference In"=w367, "Данные"=TRUE) -> ("FPGA VI Reference Out"=w366:refnum<k20>)  [unwired: 1 in, 1 out]
                    n214 = Wait (ms)(milliseconds to wait=u32 1) -> ()  [unwired: 1 out]
                  }
                  frame #3 {
                    n215 = xnode "Read/Write Control"("FPGA VI Reference In"=w370, "FRAME_REQ"=TRUE ("Данные")) -> ("FPGA VI Reference Out"=w371:refnum<k20>)  [unwired: 1 in, 1 out]
                    n216 = Wait (ms)(milliseconds to wait=u32 1) -> ()  [unwired: 1 out]
                  }
                  frame #4 {
                    n217 = xnode "Read/Write Control"("FPGA VI Reference In"=w375, "FRAME_REQ"=FALSE ("Данные")) -> ("FPGA VI Reference Out"=w374:refnum<k20>)  [unwired: 1 in, 1 out]
                    n218 = Wait (ms)(milliseconds to wait=u32 1) -> ()  [unwired: 1 out]
                  }
                  frame #5 {
                    n219 = while {
                      tunnel: w379 -> [w381]
                      tunnel: [w380] -> w378
                      stop <- w384 stop-if-true
                      n220 = xnode "Read/Write Control"("FPGA VI Reference In"=w381) -> ("FPGA VI Reference Out"=w380:refnum<k20>, "Записали адресов"=w383:u32)  [unwired: 1 in, 1 out]
                      n221 = Greater?(x=w383, y=u32 2097150) -> (0:w384:bool)
                    }
                  }
                  frame #6 {
                    n222 = xnode "Read/Write Control"("FPGA VI Reference In"=w386, "Конец анализа"=TRUE ("Данные")) -> ("FPGA VI Reference Out"=w385:refnum<k20>)  [unwired: 1 in, 1 out]
                    n223 = Wait (ms)(milliseconds to wait=u32 1) -> ()  [unwired: 1 out]
                  }
                  frame #7 {
                    n224 = xnode "Read/Write Control"("FPGA VI Reference In"=w389, "Конец анализа"=FALSE ("Данные")) -> ()  [unwired: 1 in, 2 out]
                    n225 = xnode "Read/Write Control"("FPGA VI Reference In"=w389, "Данные"=FALSE) -> ()  [unwired: 1 in, 2 out]
                    n226 = Wait (ms)(milliseconds to wait=u32 1) -> ()  [unwired: 1 out]
                  }
                }
                n227 = xnode "Invoke Method"("FPGA VI Reference In"=w346, "Number of Elements"=u32 0, "Timeout (ms)"=0) -> ("FPGA VI Reference Out"=w357:refnum<k20>, "error out"=w356:errorcluster, "Elements Remaining"=w355:u32)  [unwired: 1 in, 1 out]
                n228 = xnode "Invoke Method"("FPGA VI Reference In"=w357, "error in"=w356, "Number of Elements"=w355, "Timeout (ms)"=0) -> ("FPGA VI Reference Out"=w345:refnum<k20>)  [unwired: 3 out]
              }
              frame #1 {
                n229 = flat-sequence {
                  tunnel: w399 -> [w400]
                  tunnel: [w403] -> w398
                  tunnel: w397 -> [w403]
                  tunnel: [w402] -> w396
                  tunnel: w395 -> [w402]
                  tunnel: ["For FIFO"] -> w394
                  tunnel: [w400] -> w393
                  tunnel: w398 -> [w408]
                  tunnel: w396 -> [w407]
                  tunnel: w394 -> [w406]
                  tunnel: w393 -> [w405]
                  frame #0 {
                    # "2097152/16384"
                  }
                  frame #1 {
                    n230 = for {
                      N: w406 -> [_]
                      shift-right: [w412] -> _
                      shift-left: w408 -> [w414]
                      shift-right: [w411] -> _
                      shift-left: w407 -> [w413]
                      tunnel: w405 -> [w410]
                      tunnel: [w409] -> w404 mode=indexing
                      n231 = stacked-sequence {
                        tunnel: [_ _ _ _ w433] -> w409
                        tunnel: [w420 _ _ _ _] -> w412
                        tunnel: [w419 _ _ _ _] -> w411
                        tunnel: w414 -> [w416 _ _ _ _]
                        tunnel: w413 -> [w417 _ _ _ _]
                        tunnel: w410 -> [w415 w421 w423 w425 w432]
                        frame #0 {
                          n232 = xnode "Read/Write Control"("FPGA VI Reference In"=w415, "Нач_адр"=w416, "Кон_адр"=w417) -> ()  [unwired: 1 in, 2 out]
                          n233 = local read "32768"() -> (w418:u32)
                          n234 = Add(x=w416, y=w418) -> (x+y=w420:u32)
                          n235 = Add(x=w418, y=w417) -> (x+y=w419:u32)
                        }
                        frame #1 {
                          n236 = xnode "Read/Write Control"("FPGA VI Reference In"=w421, "Кадр на ПК"=TRUE ("HOST")) -> ()  [unwired: 1 in, 2 out]
                        }
                        frame #2 {
                          n237 = xnode "Read/Write Control"("FPGA VI Reference In"=w423, "Кадр на ПК"=FALSE ("HOST")) -> ()  [unwired: 1 in, 2 out]
                        }
                        frame #3 {
                          n238 = while {
                            tunnel: w425 -> [w426]
                            stop <- w428 stop-if-true
                            # "Записан FIFO?"
                            n239 = xnode "Read/Write Control"("FPGA VI Reference In"=w426) -> ("Записали FIFO"=w428:bool)  [unwired: 1 in, 2 out]
                            n240 = Wait (ms)(milliseconds to wait=u32 1) -> ()  [unwired: 1 out]
                          }
                        }
                        frame #4 {
                          n241 = xnode "Invoke Method"("FPGA VI Reference In"=w432, "Number of Elements"=u32 0, "Timeout (ms)"=0) -> ("FPGA VI Reference Out"=w434:refnum<k20>, "Elements Remaining"=w435:u32)  [unwired: 1 in, 2 out]
                          n242 = xnode "Invoke Method"("FPGA VI Reference In"=w434, "Number of Elements"=w435, "Timeout (ms)"=0) -> ("Data"=w433:u32[])  [unwired: 1 in, 3 out]
                        }
                      }
                    }
                    "Data" <- w404
                  }
                }
              }
            }
          }
        }
      }
      frame #1 {
        n243 = local read "Стоп"() -> (w436:bool)
      }
    }
  }
  n244 = while {
    shift-right: [w445] -> _
    shift-left: _ -> [w446]
    tunnel: w5 -> [w444]
    shift-right: ["НАДО"] -> _
    shift-left: _ -> [w440]
    stop <- w443 stop-if-true
    # "Прошиваем регистры"
    # "Если питание вновь включили, то конфигурация системного сброса, автомат, SPI"
    n245 = local read "Питание"() -> (w445:bool)
    n246 = Greater?(x=w445, y=w446) -> (0:w441:bool)
    n247 = Greater?(x="НАДО", y=w440) -> (0:w439:bool)
    n248 = Or(x=w441, y=w439) -> (x .or. y?=w442:bool)
    n249 = case shown="True" w442 {
      tunnel: w444 -> [_ w453]
      tunnel: [w447 w449] -> w443
      frame False {
        n250 = local read "Стоп"() -> (w447:bool)
      }
      frame True {
        n251 = flat-sequence {
          tunnel: [w454] -> w452
          tunnel: w453 -> [w454]
          tunnel: w452 -> [w457]
          tunnel: [w456] -> w450
          tunnel: [w459] -> w451
          tunnel: w450 -> [w459]
          tunnel: w451 -> [w464]
          tunnel: [w462] -> w448
          tunnel: w448 -> [w466]
          tunnel: [w492] -> w449
          frame #0 {
            n252 = Wait (ms)(milliseconds to wait=u32 1) -> ()  [unwired: 1 out]
          }
          frame #1 {
            n253 = xnode "Read/Write Control"("FPGA VI Reference In"=w457, "Автомат"=TRUE ("SYS_RESET")) -> ("FPGA VI Reference Out"=w456:refnum<k20>)  [unwired: 1 in, 1 out]
          }
          frame #2 {
            n254 = Wait (ms)(milliseconds to wait=u32 1) -> ()  [unwired: 1 out]
          }
          frame #3 {
            n255 = xnode "Read/Write Control"("FPGA VI Reference In"=w464, "SYS_RESET"=TRUE) -> ("FPGA VI Reference Out"=w462:refnum<k20>)  [unwired: 1 in, 1 out]
            n256 = Wait (ms)(milliseconds to wait=u32 1) -> ()  [unwired: 1 out]
          }
          frame #4 {
            n257 = for {
              N: 124 -> [_]
              tunnel: w466 -> [w467]
              i -> [w468]
              n258 = stacked-sequence {
                tunnel: w468 -> [w479 _ _ _ _]
                tunnel: w467 -> [w472 _ w482 w484 w487]
                frame #0 {
                  n259 = To Unsigned Word Integer(number=w479) -> (unsigned 16bit integer=w478:u16)
                  n260 = Index Array(array="Запись всех регистров", index=w479) -> (element=w473:u16)
                  n261 = Multiply(x=u16 256, y=w478) -> (x*y=w476:u16)
                  n262 = Add(x=u16 32768, y=w476) -> (x+y=w474:u16)
                  n263 = Add(x=w473, y=w474) -> (x+y=w471:u16)
                  n264 = Number To Boolean Array(number=w471) -> (Boolean array=w470:bool[])
                  n265 = Reverse 1D Array(array=w470) -> (reversed array=w469:bool[])
                  n266 = xnode "Read/Write Control"("FPGA VI Reference In"=w472, "SPI_IN"=w469) -> ()  [unwired: 1 in, 2 out]
                }
                frame #1 {
                  n267 = Wait (ms)(milliseconds to wait=u32 1) -> ()  [unwired: 1 out]
                }
                frame #2 {
                  n268 = xnode "Read/Write Control"("FPGA VI Reference In"=w482, "SPI"=TRUE) -> ()  [unwired: 1 in, 2 out]
                }
                frame #3 {
                  n269 = while {
                    tunnel: w484 -> [w486]
                    stop <- w485 stop-if-true
                    n270 = xnode "Read/Write Control"("FPGA VI Reference In"=w486) -> ("SPI_OFF"=w485:bool)  [unwired: 1 in, 2 out]
                  }
                }
                frame #4 {
                  n271 = xnode "Read/Write Control"("FPGA VI Reference In"=w487, "SPI"=FALSE) -> ()  [unwired: 1 in, 2 out]
                  n272 = Wait (ms)(milliseconds to wait=u32 1) -> ()  [unwired: 1 out]
                }
              }
            }
          }
          frame #5 {
            n273 = local read "Стоп"() -> (w492:bool)
            n274 = local write "СБОЙ!"(FALSE ("СБОЙ!")) -> ()
            n275 = local write "НАДО"(FALSE ("НАДО")) -> ()
            "REG_WR" <- TRUE ("Прошили регистры")
          }
        }
      }
    }
  }
  n276 = while {
    tunnel: w5 -> [_]
    shift-right: [w494] -> _
    shift-left: _ -> [w502]
    shift-right: [w495] -> _
    shift-left: _ -> [w503]
    stop <- w511 stop-if-true
    # "Это для первого образца"
    # "L"
    # "H"
    n277 = local read "COUNT"() -> (w507:u16)
    n278 = Wait (ms)(milliseconds to wait=u32 100) -> ()  [unwired: 1 out]
    n279 = local read "SPI_OUT"() -> (w504:bool[])
    n280 = Equal?(x=w507, y=u16 126) -> (x = y?=w505:bool)
    n281 = Equal?(x=w507, y=u16 127) -> (x = y?=w506:bool)
    n282 = case shown="True" w505 {
      tunnel: w504 -> [_ w517]
      tunnel: [w515 w516] -> w495
      tunnel: w503 -> [w515 _]
      frame False {
      }
      frame True {
        n283 = Boolean Array To Number(Boolean array=w517) -> (number=w516:u8)
      }
    }
    n284 = case shown="True" w506 {
      tunnel: w504 -> [_ w514]
      tunnel: [w512 w513] -> w494
      tunnel: w502 -> [w512 _]
      frame False {
      }
      frame True {
        n285 = Boolean Array To Number(Boolean array=w514) -> (number=w513:u8)
      }
    }
    n286 = Add(x=w495, y=w494) -> (x+y=w496:u8)
    n287 = local read "Стоп"() -> (w511:bool)
    n288 = Subtract(x=w496, y=u8 124) -> (x-y=w499:u8)
    n289 = To Double Precision Float(number=w499) -> (double precision float=w498:dbl)
    n290 = Multiply(x=2.4, y=w498) -> (x*y=→"T, C":dbl)
  }
  n291 = while {
    tunnel: w13 -> [w525]
    tunnel: w14 -> [w520]
    tunnel: w15 -> [w519]
    tunnel: [w524] -> _
    tunnel: [w523] -> _
    tunnel: [w522] -> _
    stop <- w518 stop-if-true
    n292 = Wait (ms)(milliseconds to wait=u32 1) -> ()  [unwired: 1 out]
    n293 = stacked-sequence {
      seq-local: ["Стоп" _] -> [_ w551]
      tunnel: w525 -> [_ w583]
      tunnel: [_ w582] -> w524
      tunnel: [_ w581] -> w523
      tunnel: [_ w580] -> w522
      tunnel: w520 -> [_ w568]
      tunnel: w519 -> [_ w556]
      tunnel: [_ w551] -> w518
      frame #0 {
      }
      frame #1 {
        w555 = T5 0 items=["Current", "Voltage"] ("measurement type")
        n294 = Not(x=w551) -> (.not. x?=w549:bool)
        n295 = Not(x=w551) -> (.not. x?=w553:bool)
        n296 = And(x=w553, y="Питание") -> (x .and. y?=w554:bool)
        n297 = And(x="Грелка", y=w549) -> (x .and. y?=w548:bool)
        n298 = call <instrlib>:"niDCPower Configure Current Limit.vi"("current limit"="REC_curlim", "channel name"="0", "instrument handle"=w556) -> ("instrument handle out"=w612:refnum<k15>)  [unwired: 7 in, 1 out]
        n299 = call <instrlib>:"niDCPower Configure Current Limit.vi"("current limit"="FPGA+REP_curlim", "channel name"="1", "instrument handle"=w556) -> ("instrument handle out"=w613:refnum<k15>)  [unwired: 7 in, 1 out]
        n300 = call <instrlib>:"niDCPower Configure Current Limit.vi"("current limit"="VDD20_curlim", "channel name"="1", "instrument handle"=w568) -> ("instrument handle out"=w614:refnum<k15>)  [unwired: 7 in, 1 out]
        n301 = call <instrlib>:"niDCPower Configure Current Limit.vi"("current limit"="VDD33_curlim", "channel name"="0", "instrument handle"=w583) -> ("instrument handle out"=w615:refnum<k15>)  [unwired: 7 in, 1 out]
        n302 = call <instrlib>:"niDCPower Configure Current Limit.vi"("current limit"="VRES_H_curlim", "channel name"="1", "instrument handle"=w583) -> ("instrument handle out"=w616:refnum<k15>)  [unwired: 7 in, 1 out]
        n303 = call <instrlib>:"niDCPower Configure Current Limit.vi"("current limit"="VDDPIX_curlim", "channel name"="0", "instrument handle"=w568) -> ("instrument handle out"=w573:refnum<k15>)  [unwired: 7 in, 1 out]
        n304 = call <instrlib>:"niDCPower Configure Current Limit.vi"("current limit"="TH_RES_curlim", "channel name"="2", "instrument handle"=w556) -> ("instrument handle out"=w562:refnum<k15>)  [unwired: 7 in, 1 out]
        n305 = call <instrlib>:"niDCPower Configure Voltage Level.vi"("voltage level"="VDD20", "channel name"="1", "instrument handle"=w614) -> ("error out"=w598:errorcluster, "instrument handle out"=w597:refnum<k15>)  [unwired: 7 in]
        n306 = call <instrlib>:"niDCPower Configure Voltage Level.vi"("voltage level"="VDD33", "channel name"="0", "instrument handle"=w615) -> ("error out"=w605:errorcluster, "instrument handle out"=w608:refnum<k15>)  [unwired: 7 in]
        n307 = call <instrlib>:"niDCPower Configure Voltage Level.vi"("voltage level"="VRES_H", "channel name"="1", "instrument handle"=w616) -> ("error out"=w606:errorcluster, "instrument handle out"=w607:refnum<k15>)  [unwired: 7 in]
        n308 = call <instrlib>:"niDCPower Configure Voltage Level.vi"("voltage level"="REC(3,3V)", "channel name"="0", "instrument handle"=w612) -> ("error out"=w588:errorcluster, "instrument handle out"=w591:refnum<k15>)  [unwired: 7 in]
        n309 = call <instrlib>:"niDCPower Configure Voltage Level.vi"("voltage level"="FPGA+REP(6V)", "channel name"="1", "instrument handle"=w613) -> ("error out"=w589:errorcluster, "instrument handle out"=w590:refnum<k15>)  [unwired: 7 in]
        n310 = call <instrlib>:"niDCPower Configure Voltage Level.vi"("voltage level"="VDDPIX", "channel name"="0", "instrument handle"=w573) -> ("error out"=w577:errorcluster, "instrument handle out"=w578:refnum<k15>)  [unwired: 7 in]
        n311 = call <instrlib>:"niDCPower Configure Voltage Level.vi"("voltage level"="TH_RES", "channel name"="2", "instrument handle"=w562) -> ("error out"=w565:errorcluster, "instrument handle out"=w564:refnum<k15>)  [unwired: 7 in]
        n312 = call <instrlib>:"niDCPower Configure Output Enabled.vi"("error in (no error)"=w598, "output enabled"=w554, "channel name"="1", "instrument handle"=w597) -> ("error out"=w636:errorcluster, "instrument handle out"=w631:refnum<k15>)  [unwired: 6 in]
        n313 = call <instrlib>:"niDCPower Configure Output Enabled.vi"("error in (no error)"=w605, "output enabled"=w554, "channel name"="0", "instrument handle"=w608) -> ("error out"=w633:errorcluster, "instrument handle out"=w632:refnum<k15>)  [unwired: 6 in]
        n314 = call <instrlib>:"niDCPower Configure Output Enabled.vi"("error in (no error)"=w606, "output enabled"=w554, "channel name"="1", "instrument handle"=w607) -> ("error out"=w634:errorcluster, "instrument handle out"=w635:refnum<k15>)  [unwired: 6 in]
        n315 = call <instrlib>:"niDCPower Configure Output Enabled.vi"("error in (no error)"=w588, "output enabled"=w554, "channel name"="0", "instrument handle"=w591) -> ("error out"=w623:errorcluster, "instrument handle out"=w622:refnum<k15>)  [unwired: 6 in]
        n316 = call <instrlib>:"niDCPower Configure Output Enabled.vi"("error in (no error)"=w589, "output enabled"=w554, "channel name"="1", "instrument handle"=w590) -> ("error out"=w624:errorcluster, "instrument handle out"=w625:refnum<k15>)  [unwired: 6 in]
        n317 = call <instrlib>:"niDCPower Configure Output Enabled.vi"("error in (no error)"=w577, "output enabled"=w554, "channel name"="0", "instrument handle"=w578) -> ("error out"=w569:errorcluster, "instrument handle out"=w570:refnum<k15>)  [unwired: 6 in]
        n318 = call <instrlib>:"niDCPower Configure Output Enabled.vi"("error in (no error)"=w565, "output enabled"=w548, "channel name"="2", "instrument handle"=w564) -> ("error out"=w560:errorcluster, "instrument handle out"=w559:refnum<k15>)  [unwired: 6 in]
        n319 = call <instrlib>:"niDCPower Measure.vi"("error in (no error)"=w623, "measurement type"=w555, "channel name"="0", "instrument handle"=w622) -> ("measurement"=w529:dbl, "instrument handle out"=w582:refnum<k15>)  [unwired: 5 in, 1 out]
        "REC_cur" <- w529
        n320 = call <instrlib>:"niDCPower Measure.vi"("error in (no error)"=w624, "measurement type"=w555, "channel name"="1", "instrument handle"=w625) -> ("measurement"=w540:dbl)  [unwired: 5 in, 2 out]
        "FPGA+REP_cur" <- w540
        n321 = call <instrlib>:"niDCPower Measure.vi"("error in (no error)"=w636, "measurement type"=w555, "channel name"="1", "instrument handle"=w631) -> ("measurement"=w534:dbl, "instrument handle out"=w581:refnum<k15>)  [unwired: 5 in, 1 out]
        "VDD20_cur" <- w534
        n322 = call <instrlib>:"niDCPower Measure.vi"("error in (no error)"=w569, "measurement type"=w555, "channel name"="0", "instrument handle"=w570) -> ("measurement"=w536:dbl)  [unwired: 5 in, 2 out]
        "VDDPIX_cur" <- w536
        n323 = call <instrlib>:"niDCPower Measure.vi"("error in (no error)"=w560, "measurement type"=w555, "channel name"="2", "instrument handle"=w559) -> ("measurement"=w538:dbl)  [unwired: 5 in, 2 out]
        "TH_RES_cur" <- w538
        n324 = call <instrlib>:"niDCPower Measure.vi"("error in (no error)"=w633, "measurement type"=w555, "channel name"="0", "instrument handle"=w632) -> ("measurement"=w533:dbl, "instrument handle out"=w580:refnum<k15>)  [unwired: 5 in, 1 out]
        "VDD33_cur" <- w533
        n325 = call <instrlib>:"niDCPower Measure.vi"("error in (no error)"=w634, "measurement type"=w555, "channel name"="1", "instrument handle"=w635) -> ("measurement"=w531:dbl)  [unwired: 5 in, 2 out]
        "VRES_H_cur" <- w531
        n326 = Multiply(x=w534, y=1000.0) -> (x*y=→"Waveform Chart 6":dbl)
        n327 = Multiply(x=w529, y=1000.0) -> (x*y=→"Waveform Chart 5":dbl)
        n328 = Multiply(x=w540, y=1000.0) -> (x*y=→"Waveform Chart 2":dbl)
        n329 = Multiply(x=w533, y=1000.0) -> (x*y=→"Waveform Chart 7":dbl)
        n330 = Multiply(x=w538, y=1000.0) -> (x*y=→"Waveform Chart 3":dbl)
        n331 = Multiply(x=w536, y=1000.0) -> (x*y=→"Waveform Chart 4":dbl)
        n332 = Multiply(x=w531, y=1000.0) -> (x*y=→"Waveform Chart 9":dbl)
      }
    }
  }
  n333 = while {
    tunnel: w5 -> [w639]
    stop <- w640 stop-if-true
    n334 = local read "Стоп"() -> (w642:bool)
    n335 = xnode "Read/Write Control"("FPGA VI Reference In"=w639, "2"="2", "1"="1", "REQ_1"="REQ_1", "REQ_2"="REQ_2", "-1_прием"="-1_прием", "Стоп"=w642, "9_прием"="9_прием") -> ("D9"=→"D9":bool[], "CONTROL"=→"CONTROL":bool[], "D1"=→"D1":bool[], "Записали адресов"=→"Записали адресов":u32)  [unwired: 1 in, 2 out]
    n336 = Wait (ms)(milliseconds to wait=u32 1) -> ()  [unwired: 1 out]
    n337 = local read "Стоп"() -> (w640:bool)
  }
  n338 = while {
    shift-right: ["SAVE"] -> _
    shift-left: _ -> [w664]
    stop <- w666 stop-if-true
    n339 = local read "Запись всех регистров"() -> (w658:u16[])
    n340 = Greater?(x="SAVE", y=w664) -> (0:w663:bool)
    n341 = Index Array(array=w658, index=43) -> (element=w661:u16)
    n342 = Multiply(x=w661, y=6604800.0) -> (x*y=w660:dbl)
    n343 = Add(x=w660, y=221880.0) -> (x+y=w659:dbl)
    n344 = Divide(x=w659, y=1000000.0) -> (x/y=w653:dbl)
    "Тнак, мс" <- w653
    n345 = case shown="True" w663 {
      tunnel: w653 -> [_ w685]
      frame False {
      }
      frame True {
        w683 = i16 1 ("precision (6)")
        w686 = i16 0 ("precision (6)")
        w681 = "_"
        n346 = local read "Номер образца"() -> (w669:string)
        n347 = local read "Температура"() -> (w672:string)
        n348 = local read "T, C"() -> (w682:dbl)
        n349 = Concatenate Strings("Темп. = " ("string"), w672) -> (w670:string)
        n350 = Concatenate Strings("Образец_" ("string"), w669) -> (w667:string)
        n351 = Get Date/Time In Seconds() -> (seconds since 1Jan1904=w701:timestamp)
        n352 = Number To Fractional String(number=w685, width (-)=w686, precision (6)=w686) -> (F-format string=w684:string)  [unwired: 1 in]
        n353 = Number To Fractional String(number=w682, width (-)=w683, precision (6)=w683) -> (F-format string=w679:string)  [unwired: 1 in]
        n354 = Format Date/Time String(time format string (%c)="%H.%M.%S", seconds (now)=w701) -> (date/time string=w705:string)  [unwired: 1 in]
        n355 = Select(t="Светло", s="Светлый (T)\nТемный (F)", f="Темно") -> (s? t:f=w702:string)
        n356 = Build Path(base path="Frames", name or relative path=w667) -> (appended path=w696:path)
        n357 = call <vilib>:"Check if File or Folder Exists.vi"("path"=w696) -> ("file or folder exists?"=w695:bool, "dup path"=w694:path)  [unwired: 8 in, 1 out]
        n358 = case shown="False" w695 {
          tunnel: w694 -> [w714 w715]
          tunnel: [w713 w715] -> w674
          frame False {
            n359 = Create Folder(path (use dialog)=w714) -> (created path=w713:path)  [unwired: 2 in, 2 out]
          }
          frame True {
          }
        }
        n360 = Build Path(base path=w674, name or relative path=w670) -> (appended path=w675:path)
        n361 = call <vilib>:"Check if File or Folder Exists.vi"("path"=w675) -> ("file or folder exists?"=w676:bool, "dup path"=w677:path)  [unwired: 8 in, 1 out]
        n362 = case shown="False" w676 {
          tunnel: w677 -> [w708 w709]
          tunnel: [w707 w709] -> w673
          frame False {
            n363 = Create Folder(path (use dialog)=w708) -> (created path=w707:path)  [unwired: 2 in, 2 out]
          }
          frame True {
          }
        }
        n364 = Build Path(base path=w673, name or relative path=w702) -> (appended path=w697:path)
        n365 = call <vilib>:"Check if File or Folder Exists.vi"("path"=w697) -> ("file or folder exists?"=w698:bool, "dup path"=w699:path)  [unwired: 8 in, 1 out]
        n366 = case shown="False" w698 {
          tunnel: w699 -> [w711 w712]
          tunnel: [w710 w712] -> w703
          frame False {
            n367 = Create Folder(path (use dialog)=w711) -> (created path=w710:path)  [unwired: 2 in, 2 out]
          }
          frame True {
          }
        }
        n368 = local read "Image"() -> (w688:T1)
        n369 = Concatenate Strings(w705, w681, "ПРИМЕЧАНИЕ", w681, "Тн(мс)=" ("string"), w684, w681, "Темп(гр)=" ("string"), w679, ".tiff" ("element")) -> (w704:string)
        n370 = Build Path(base path=w703, name or relative path=w704) -> (appended path=w700:path)
        n371 = call-poly "IMAQ Write File 2"("File Path"=w700, "Image"=w688) -> ()  [unwired: 8 in, 2 out]
      }
    }
    n372 = Wait (ms)(milliseconds to wait=u32 1) -> ()  [unwired: 1 out]
    n373 = local read "Стоп"() -> (w666:bool)
  }
  n374 = call "IMAQ Create"("Image Name"="CMV", "Image Type"=w3) -> ("New Image"=w2:T1)  [unwired: 3 in, 1 out]
  n375 = while {
    tunnel: w2 -> [w717]
    stop <- w724 stop-if-true
    w721 = 2048
    n376 = local read "Data"() -> (w719:u32[][])
    n377 = Reshape Array(w719, 2097152 ("dimension size")) -> (w722:u32[])
    n378 = for {
      N: w721 -> [_]
      tunnel: [w734] -> w723 mode=indexing
      shift-right: [w732] -> _
      shift-left: w722 -> [w740]
      w733 = 1024 ("length")
      n379 = Delete From Array(array=w740, length=w733, index=0) -> (deleted portion=w738:u32[], array with subset deleted=w732:u32[])
      n380 = for {
        N: w733 -> [_]
        tunnel: w738 -> [w748] mode=indexing
        tunnel: [w743] -> w737 mode=indexing
        tunnel: [w742] -> w735 mode=indexing
        # "D9"
        # "D1"
        n381 = Number To Boolean Array(number=w748) -> (Boolean array=w747:bool[])
        n382 = Delete From Array(array=w747, length=10, index=0) -> (deleted portion=w744:bool[], array with subset deleted=w741:bool[])
        n383 = Boolean Array To Number(Boolean array=w744) -> (number=w743:u32)
        n384 = Boolean Array To Number(Boolean array=w741) -> (number=w742:u32)
      }
      n385 = Insert Into Array(array=w737, index=1024, new element=w735) -> (w734:u32[])
    }
    n386 = local read "Стоп"() -> (w724:bool)
    n387 = for {
      N: w721 -> [_]
      tunnel: w723 -> [w727] mode=indexing
      tunnel: w721 -> [w726]
      tunnel: [w725] -> w718 mode=indexing
      n388 = for {
        N: w726 -> [_]
        tunnel: w727 -> [w730] mode=indexing
        tunnel: [w731] -> w725 mode=indexing
        n389 = Multiply(x=w730, y=u32 64) -> (x*y=w728:u32)
        n390 = Bundle(w728, w728, w728, w728) -> (w731:cluster{u32, u32, u32, u32})  [unwired: 1 in]
      }
    }
    n391 = call "IMAQ ArrayToColorImage"("Image"=w717, "Image Pixels (U64)"=w718) -> ("Image Out"=→"Image Out":T1)  [unwired: 3 in, 1 out]
  }
  n392 = while {
    stop <- w750 stop-if-true
    n393 = Wait (ms)(milliseconds to wait=u32 1) -> ()  [unwired: 1 out]
    n394 = local read "Image Out"() -> (→"Image":T1)
    n395 = local read "Стоп"() -> (w750:bool)
  }
  n396 = xnode "Invoke Method"("FPGA VI Reference In"=w11) -> ()  [unwired: 1 in, 2 out]
